vi "Generate Trace for New Network Endpoint Server.vi"(9 "Port":string, 10 "IPs or Stream Names":string[](array[string])) -> ()   [LabVIEW 2020]
doc: "Generates a DETT User Generated Trace for a network endpoint being newly launched."
uses:
  <resource>/AFDebug/AF Debug.lvlib
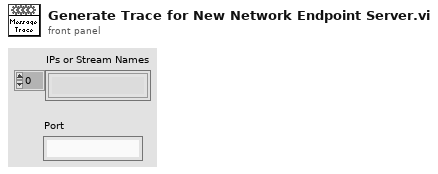
[diagram p1: front panel]
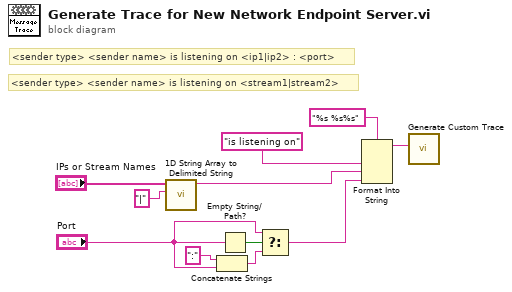
[diagram p0: block diagram]
diagram:
  # "<sender type> <sender name> is listening on <ip1|ip2> : <port>"
  # "<sender type> <sender name> is listening on <stream1|stream2>"
  n1 = call-poly <vilib>:"1D String Array to Delimited String.vi"("delimiter"="|", "string array"="IPs or Stream Names") -> ("delimited string"=w8:string)  [unwired: 9 in]
  n2 = Concatenate Strings(":" ("string"), "Port") -> (w3:string)
  n3 = Empty String/Path?(string/path="Port") -> (empty?=w4:bool)
  n4 = Select(t="Port", s=w4, f=w3) -> (s? t:f=w2:string)
  n5 = Format Into String(format string="%s %s%s", "is listening on" ("input 3"), w8, w2) -> (resulting string=w6:string)  [unwired: 2 in, 1 out]
  n6 = call <resource>:"Generate Custom Trace.vi"("Custom Action"=w6) -> ()  [unwired: 11 in]
